vi "登录FGV.vi"(7 "枚举":enum16{"init", "quit", "read", "wirte"}(ring), 11 "wirte":T1) -> (3 "wirte 2":T1)   [LabVIEW 2018, in "login.lvlib"]
uses:
  login.lvlib
  <vilib>/Utility/xml.llb/Read From XML File(string).vi
  <vilib>/Utility/xml.llb/Write to XML File(string).vi
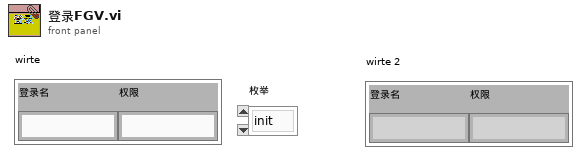
[diagram p1: front panel]
types:
  T1 = typedef "login.lvlib/登录蔟.ctl" = cluster{"登录名":string, "权限":string}
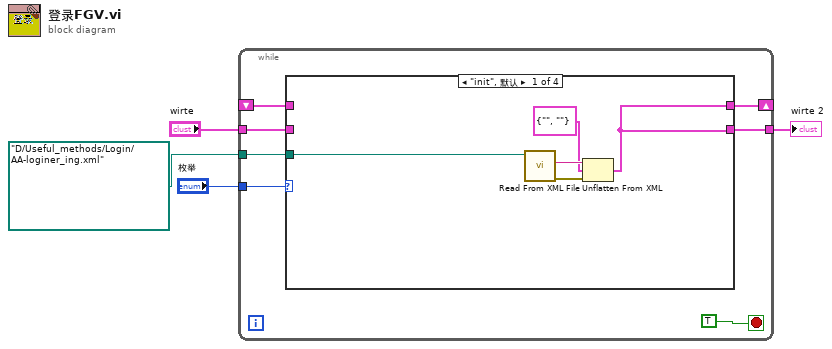
[diagram p0: block diagram]
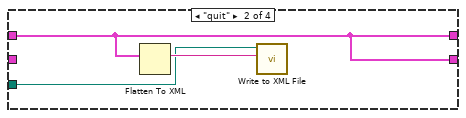
[diagram p2: hidden frame]
diagram:
  n1 = while {
    tunnel: "枚举" -> [w9]
    shift-right: [w8] -> _
    shift-left: _ -> [w10]
    tunnel: "wirte" -> [w7]
    tunnel: [w6] -> w2
    tunnel: path "D:/Useful_methods/Login/AA-loginer_ing.xml" ("路径") -> [w5]
    stop <- TRUE stop-if-true
    n2 = case shown="\"init\", 默认" w9 {
      tunnel: w10 -> [_ w18 w20 _]
      tunnel: [w13 w18 w20 w21] -> w8
      tunnel: w7 -> [_ _ _ w21]
      tunnel: [w13 w18 w20 w21] -> w6
      tunnel: w5 -> [w12 w17 _ _]
      frame "init", Default {
        n3 = call-poly <vilib>:"Read From XML File.vi"("XML File Path"=w12) -> ("error out"=w16:errorcluster, "XML Elements"=w15:string)  [unwired: 8 in, 1 out]
        n4 = Unflatten From XML(xml string=w15, type=T1 {"登录名"="", "权限"=""} ("wirte 2"), error in (no error)=w16) -> (value=w13:T1)  [unwired: 1 out]
      }
      frame "quit" {
        n5 = Flatten To XML(anything=w18) -> (xml string=w19:string)
        n6 = call-poly <vilib>:"Write to XML File.vi"("XML Input"=w19, "XML File Path"=w17) -> ()  [unwired: 7 in, 3 out]
      }
      frame "read" {
      }
      frame "wirte" {
      }
    }
  }
  "wirte 2" <- w2
